vi "Caller.vi"(11 "error in":errorcluster) -> (4 "Out":dbl, 15 "error out":errorcluster)   [LabVIEW 2026]
doc: "Issue 136 subVI example: calls Sub.vi with X wired and Result read."
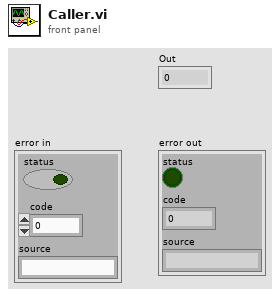
[diagram p1: front panel]
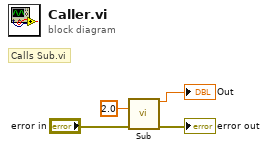
[diagram p0: block diagram]
diagram:
  # "Calls Sub.vi"
  n1 = call "Sub.vi"("X"=2.0, "error in"="error in") -> ("Result"=→"Out":dbl, "error out"=→"error out":errorcluster)  [unwired: 12 in]
